vi "PathPlanner_PathConstraints_Equals.vi"(9 "Other PathPlannerConstraints":T1={"MaxVelocityMps;"=0.0, "MaxAccelerationMpsSq;"=0.0, "MaxAngularVelRadPsEc;"=0.0, "MaxAngularAccRadPSecSq"=0.0, "Exists"=FALSE, "Unlimited"=FALSE, "NominalVoltageVolts"=12.0}, 11 "PathPlannerConstraints":T1={"MaxVelocityMps;"=0.0, "MaxAccelerationMpsSq;"=0.0, "MaxAngularVelRadPsEc;"=0.0, "MaxAngularAccRadPSecSq"=0.0, "Exists"=FALSE, "Unlimited"=FALSE, "NominalVoltageVolts"=12.0}) -> (3 "Equal":bool)   [LabVIEW 2019, in "PathPlanner24.lvlib"]
doc: "Determines if two Path Constraints definitions are nearly identical. The values have to be within 0.001 of eah other.\n\nInputs:\n - PathPlannerConstraints - cluster - definition of path constraints\n - OtherPathPlannerConstraints - cluster - definition of seond path constraints for comparision\n\nOutputs:\n - Equal - boolean - TRUE indicates the provided definitions are nearly identical."
uses:
  PathPlanner24.lvlib
  TypeDef/PathPlannerPathConstraints.ctl
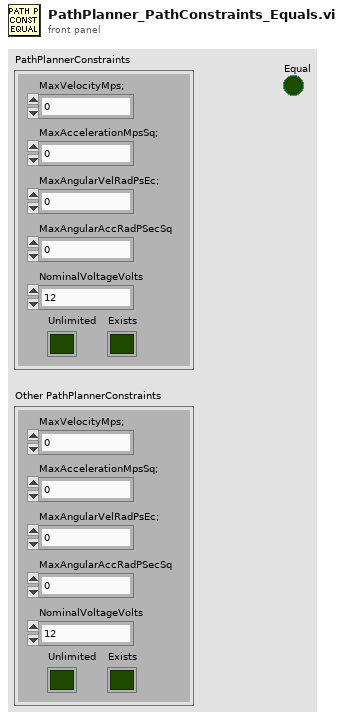
[diagram p1: front panel]
types:
  T1 = typedef "PathPlanner24.lvlib/PathPlannerPathConstraints.ctl" = cluster{"MaxVelocityMps;":dbl, "MaxAccelerationMpsSq;":dbl, "MaxAngularVelRadPsEc;":dbl, "MaxAngularAccRadPSecSq":dbl, "Exists":bool, "Unlimited":bool, "NominalVoltageVolts":dbl}
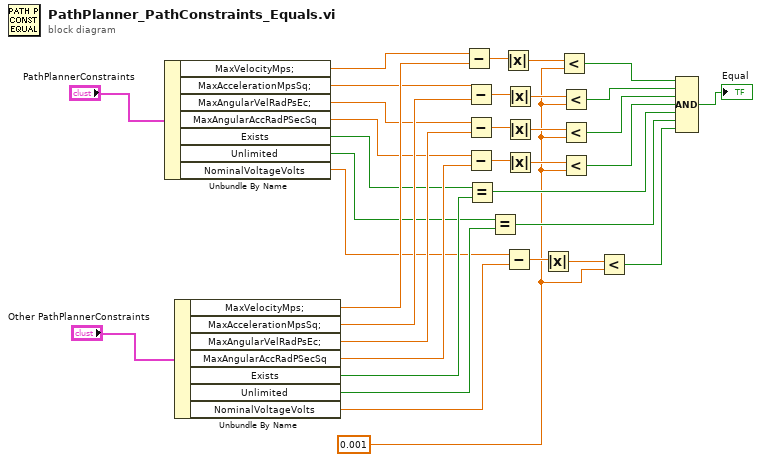
[diagram p0: block diagram]
diagram:
  w2 = 0.001 ("y")
  n1 = Unbundle By Name("PathPlannerConstraints") -> ("MaxVelocityMps;"=w33:dbl, "MaxAccelerationMpsSq;"=w23:dbl, "MaxAngularVelRadPsEc;"=w21:dbl, "MaxAngularAccRadPSecSq"=w19:dbl, "Exists"=w12:bool, "Unlimited"=w9:bool, "NominalVoltageVolts"=w4:dbl)
  n2 = Unbundle By Name("Other PathPlannerConstraints") -> ("MaxVelocityMps;"=w32:dbl, "MaxAccelerationMpsSq;"=w22:dbl, "MaxAngularVelRadPsEc;"=w20:dbl, "MaxAngularAccRadPSecSq"=w18:dbl, "Exists"=w11:bool, "Unlimited"=w8:bool, "NominalVoltageVolts"=w3:dbl)
  n3 = Subtract(x=w33, y=w32) -> (x-y=w31:dbl)
  n4 = Subtract(x=w23, y=w22) -> (x-y=w29:dbl)
  n5 = Subtract(x=w21, y=w20) -> (x-y=w27:dbl)
  n6 = Subtract(x=w19, y=w18) -> (x-y=w25:dbl)
  n7 = Equal?(x=w12, y=w11) -> (x = y?=w10:bool)
  n8 = Equal?(x=w9, y=w8) -> (x = y?=w7:bool)
  n9 = Absolute Value(x=w31) -> (abs(x)=w30:dbl)
  n10 = Subtract(x=w4, y=w3) -> (x-y=w6:dbl)
  n11 = Absolute Value(x=w29) -> (abs(x)=w28:dbl)
  n12 = Absolute Value(x=w27) -> (abs(x)=w26:dbl)
  n13 = Absolute Value(x=w25) -> (abs(x)=w24:dbl)
  n14 = Absolute Value(x=w6) -> (abs(x)=w5:dbl)
  n15 = Less?(x=w30, y=w2) -> (x < y?=w17:bool)
  n16 = Less?(x=w28, y=w2) -> (x < y?=w16:bool)
  n17 = Less?(x=w26, y=w2) -> (x < y?=w15:bool)
  n18 = Less?(x=w24, y=w2) -> (x < y?=w14:bool)
  n19 = Less?(x=w5, y=w2) -> (x < y?=w1:bool)
  n20 = Compound Arithmetic op=AND(w17, w16, w15, w14, w10, w7, w1) -> (→"Equal":bool)
